vi "set TurnTable Parameter.vi"(8 "error in (no error)":errorcluster, 10 "Turn Table Info":T1 {"Target Angle" min=0.0 max=360.0}, 11 "ETS_EM2090 in":refnum<class "ETS_EM2090.lvclass">) -> (0 "error out":errorcluster, 3 "ETS_EM2090 out":refnum<class "ETS_EM2090.lvclass">)   [LabVIEW 2023, in "Turn Table and Mast.lvlib" / "ETS_EM2090.lvclass"]
uses:
  ETS_EM2090.lvclass
  ETS_EM2090.lvclass/ETS_EM2090.ctl
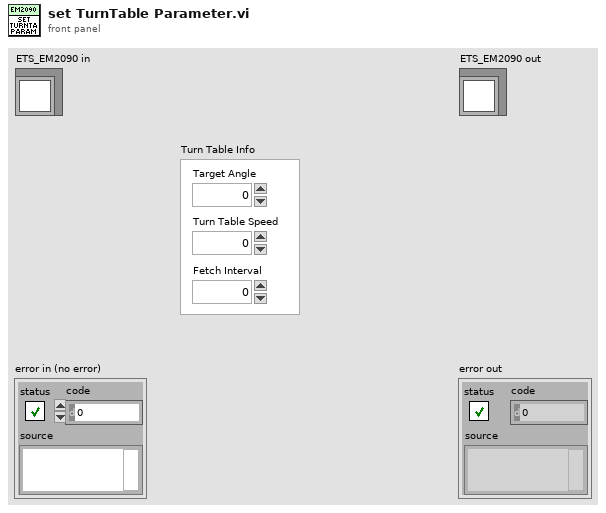
[diagram p1: front panel]
types:
  T1 = cluster{"Target Angle":dbl, "Turn Table Speed":i32, "Fetch Interval":i32}
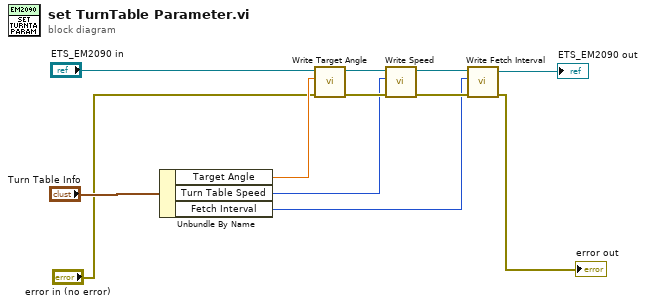
[diagram p0: block diagram]
diagram:
  n1 = Unbundle By Name("Turn Table Info") -> ("Target Angle"=w10:dbl, "Turn Table Speed"=w7:i32, "Fetch Interval"=w4:i32)
  n2 = call "Write Target Angle.vi"("error in (no error)"="error in (no error)", "Target Angle"=w10, "ETS_EM2090 in"="ETS_EM2090 in") -> ("error out"=w8:errorcluster, "ETS_EM2090 out"=w9:refnum<class "ETS_EM2090.lvclass">)  [unwired: 7 in]
  n3 = call "Write Speed.vi"("error in (no error)"=w8, "Speed"=w7, "ETS_EM2090 in"=w9) -> ("error out"=w5:errorcluster, "ETS_EM2090 out"=w6:refnum<class "ETS_EM2090.lvclass">)  [unwired: 7 in]
  n4 = call "Write Fetch Interval.vi"("error in (no error)"=w5, "Fetch Interval"=w4, "ETS_EM2090 in"=w6) -> ("error out"=→"error out":errorcluster, "ETS_EM2090 out"=→"ETS_EM2090 out":refnum<class "ETS_EM2090.lvclass">)  [unwired: 7 in]
